vi "Move.vi"(8 "error in":errorcluster, 9 "Target":path, 10 "Source":path, 11 "File Manager in":refnum<class "File Manager.lvclass">) -> (0 "error out":errorcluster, 3 "File Manager out":refnum<class "File Manager.lvclass">)   [LabVIEW 2026, in "File Manager.lvclass"]
doc: "Move (aka rename) source to target."
uses:
  File Manager.lvclass
  File Manager.lvclass/File Manager.ctl
  Interfaces/ILogger/ILogger Messages/Log Msg/Log Msg.lvclass/Log Msg.ctl
  <vilib>/ActorFramework/Message Enqueuer/Message Enqueuer.lvclass/Message Enqueuer.ctl
  <vilib>/ActorFramework/Message Enqueuer/Enqueue.vi
  Interfaces/ILogger/ILogger Messages/Log Msg/Log Msg.lvclass
  <userlib>/_OpenG.lib/file/file.llb/File Exists - Scalar__ogtk.vi
  <vilib>/ActorFramework/Message Priority Queue/Priority Enqueue.vi
  <userlib>/_OpenG.lib/file/file.llb/openg_file.lvlib
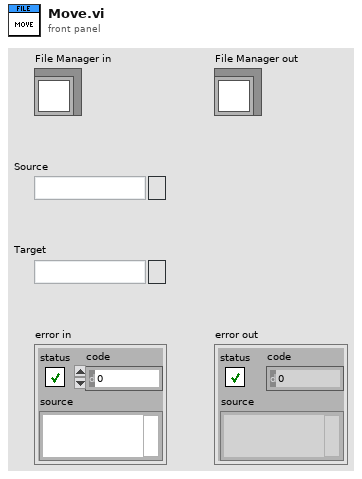
[diagram p1: front panel]
types:
  T1 = typedef "Log Entry--cluster.ctl" = cluster{"Time":timestamp, "Message":string}
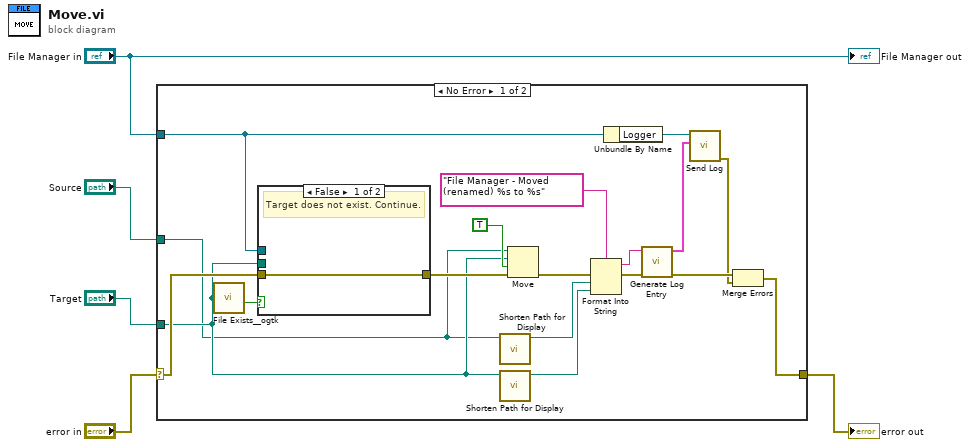
[diagram p0: block diagram]
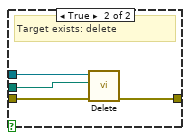
[diagram p2: hidden frame]
diagram:
  n1 = case shown="No Error" "error in" {
    selector: "error in" -> [w17 w29]
    tunnel: [w19 w29] -> w5
    tunnel: "Target" -> [w8 _]
    tunnel: "File Manager in" -> [w7 _]
    tunnel: "Source" -> [w6 _]
    frame No Error {
      n2 = call-poly <userlib>:"File Exists__ogtk.vi"("file path"=w8) -> ("exists"=w10:bool)  [unwired: 6 in, 1 out]
      n3 = case shown="False" w10 {
        tunnel: w8 -> [_ w25]
        tunnel: w17 -> [w24 w28]
        tunnel: [w24 w27] -> w23
        tunnel: w7 -> [_ w26]
        frame False {
          # "Target does not exist. Continue."
        }
        frame True {
          # "Target exists: delete"
          n4 = call-dynamic "Delete.vi"("error in"=w28, "Path"=w25, "File Manager in"=w26) -> ("error out"=w27:errorcluster)  [unwired: 7 in, 1 out]
        }
      }
      n5 = call "Shorten Path for Display.vi"("Path"=w6) -> ("Shortened Path"=w11:path)  [unwired: 10 in]
      n6 = call "Shorten Path for Display.vi"("Path"=w8) -> ("Shortened Path"=w12:path)  [unwired: 10 in]
      n7 = Move(source path=w6, error in=w23, 9:TRUE ("overwrite (F)"), 10:w8) -> (error out=w21:errorcluster)  [unwired: 1 in, 2 out]
      n8 = Format Into String(format string="File Manager - Moved (renamed) %s to %s", error in=w21, w11, w12) -> (resulting string=w14:string, error out=w22:errorcluster)  [unwired: 1 in]
      n9 = Unbundle By Name(w7) -> ("Logger"=w9:refnum<class "Message Enqueuer.lvclass">)
      n10 = call "Generate Log Entry.vi"("error in"=w22, "Message"=w14) -> ("error out"=w20:errorcluster, "Log Entry"=w13:T1)  [unwired: 8 in]
      n11 = call "Send Log.vi"("Log Entry"=w13, "Message Enqueuer"=w9) -> ("error out"=w18:errorcluster)  [unwired: 8 in, 1 out]
      n12 = Merge Errors(w20, w18) -> (w19:errorcluster)
    }
    frame Error {
      # "Pass error without further action."
    }
  }
  "error out" <- w5
  "File Manager out" <- "File Manager in"
